vi "Test_Time_Update.vi"(8 "error in (no error) 2":errorcluster, 11 "Write":string) -> (0 "error in (no error) 3":errorcluster)   [LabVIEW 2021]
uses:
  Template/Main_VI/Control/Ini.ctl
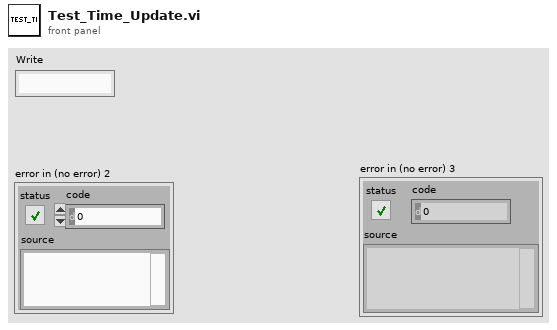
[diagram p1: front panel]
types:
  T1 = typedef "Ini.ctl" = enum16{"Write", "Read"}
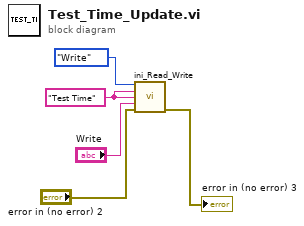
[diagram p0: block diagram]
diagram:
  w4 = "Test Time" ("Write Section")
  n1 = call "ini_Read_Write.vi"(0:Ini."Write", "Write Section"=w4, "Write key"=w4, "Write"="Write", "error in (no error) 2"="error in (no error) 2") -> ("error in (no error) 3"=→"error in (no error) 3":errorcluster)  [unwired: 9 in, 1 out]
